vi "Generate Filename.vi"(8 "error in":errorcluster, 10 "Folder":path, 11 "ILabVIEW File in":refnum<class "ILabVIEW File.lvclass">) -> (0 "error out":errorcluster, 2 "File Path":path, 3 "ILabVIEW File out":refnum<class "ILabVIEW File.lvclass">)   [LabVIEW 2026, in "ILabVIEW File.lvclass"]
doc: "This VI generates a file path suitable for saving files based on the provided folder and the implementing classes properties."
uses:
  ILabVIEW File.lvclass
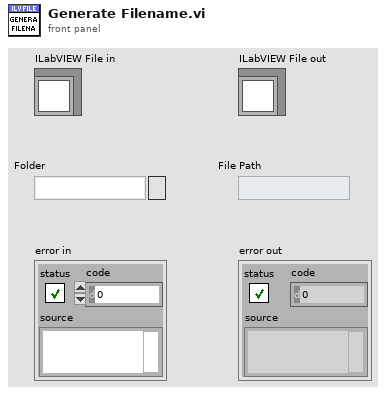
[diagram p1: front panel]
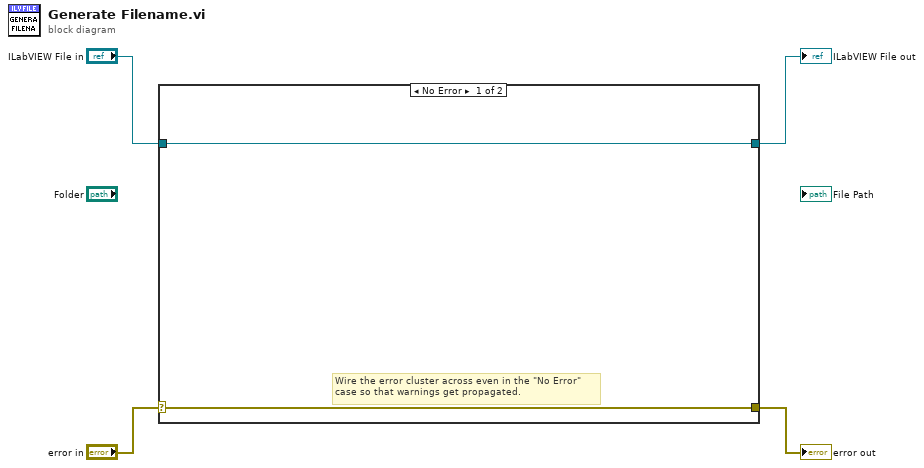
[diagram p0: block diagram]
diagram:
  n1 = case shown="No Error" "error in" {
    selector: "error in" -> [w6 w8]
    tunnel: [w6 w8] -> w3
    tunnel: [w5 w7] -> w1
    tunnel: "ILabVIEW File in" -> [w5 w7]
    frame No Error {
      # "Wire the error cluster across even in the \"No Error\"\ncase so that warnings get propagated."
    }
    frame Error {
    }
  }
  "error out" <- w3
  "ILabVIEW File out" <- w1
